vi "Read Protocol Characters.vi"(8 "error in (no error)":errorcluster, 11 "3D Controller in":refnum<class "3D Controller.lvclass">) -> (0 "error out":errorcluster, 2 "Protocol Characters":T1, 3 "3D Controller out":refnum<class "3D Controller.lvclass">)   [LabVIEW 2023, in "FCC 3D Controller for BS.lvlib" / "3D Controller.lvclass"]
uses:
  3D Controller.lvclass
  3D Controller.lvclass/3D Controller.ctl
  Type Definition/TYPE Protocol Char of Command.ctl
  FCC 3D Controller for BS.lvlib
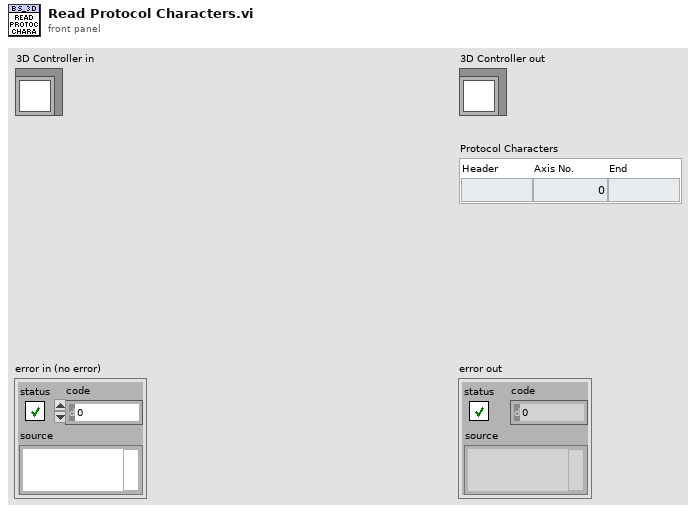
[diagram p1: front panel]
types:
  T1 = typedef "FCC 3D Controller for BS.lvlib/TYPE Protocol Char of Command.ctl" = cluster{"Header":string, "Axis No.":i32, "End":string}
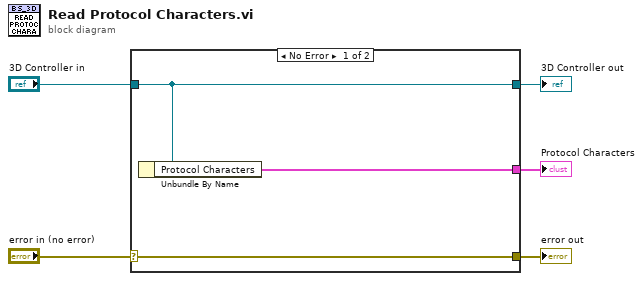
[diagram p0: block diagram]
diagram:
  n1 = case shown="No Error" "error in (no error)" {
    selector: "error in (no error)" -> [w8 w9]
    tunnel: [w8 w9] -> w4
    tunnel: [w7 w10] -> w2
    tunnel: "3D Controller in" -> [w7 w10]
    tunnel: [w6 _] -> w1
    frame No Error {
      n2 = Unbundle By Name(w7) -> ("Protocol Characters"=w6:T1)
    }
    frame Error {
    }
  }
  "error out" <- w4
  "3D Controller out" <- w2
  "Protocol Characters" <- w1
